vi "Parse Category from Frame Name.vi"(11 "Frame Name":string) -> (2 "is a Category?":bool, 3 "Category Name":string)   [LabVIEW 2020, in "JKI State Machine API.lvlib" / "JKI SM.lvclass"]
uses:
  JKI SM.lvclass
  <userlib>/_OpenG.lib/string/string.llb/Trim Whitespace (String)__ogtk.vi
  JKI SM.lvclass/JKI SM.ctl
  <userlib>/_OpenG.lib/string/string.llb/openg_string.lvlib
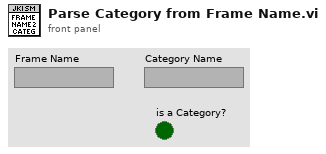
[diagram p1: front panel]
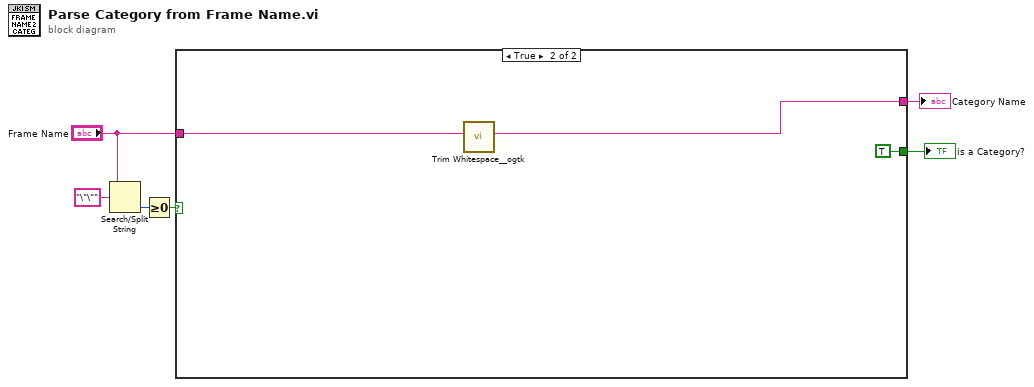
[diagram p0: block diagram]
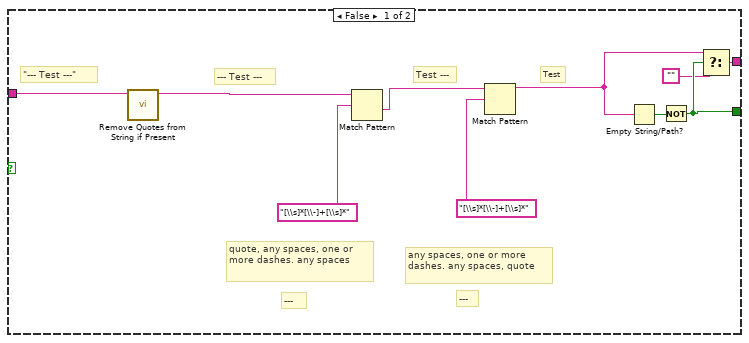
[diagram p2: hidden frame]
diagram:
  n1 = Search/Split String(string="Frame Name", search string/char (-)="\"\"") -> (offset of match=w1:i32)  [unwired: 1 in, 2 out]
  n2 = Greater Or Equal To 0?(x=w1) -> (x >= 0?=w2:bool)
  n3 = case shown="True" w2 {
    tunnel: [w11 TRUE] -> w6
    tunnel: [w9 w17] -> w5
    tunnel: "Frame Name" -> [w7 w19]
    frame False {
      # "--- Test ---"
      # "---"
      # "---"
      # "Test"
      # "Test ---"
      # "\"--- Test ---\""
      # "any spaces, one or more dashes. any spaces, quote"
      # "quote, any spaces, one or more dashes. any spaces"
      n4 = call "Remove Quotes from String if Present.vi"("String"=w7) -> ("String with Quotes Removed"=w8:string)  [unwired: 10 in]
      n5 = Match Pattern(string=w8, regular expression="[\\s]*[\\-]+[\\s]*") -> (after substring=w14:string)  [unwired: 1 in, 3 out]
      n6 = Match Pattern(string=w14, regular expression="[\\s]*[\\-]+[\\s]*") -> (before substring=w13:string)  [unwired: 1 in, 3 out]
      n7 = Empty String/Path?(string/path=w13) -> (empty?=w16:bool)
      n8 = Not(x=w16) -> (.not. x?=w11:bool)
      n9 = Select(t=w13, s=w11, f="") -> (s? t:f=w9:string)
    }
    frame True {
      n10 = call-poly <userlib>:"Trim Whitespace__ogtk.vi"("String in"=w19) -> ("String out"=w17:string)  [unwired: 6 in]
    }
  }
  "is a Category?" <- w6
  "Category Name" <- w5
